vi "Step Response.vi"() -> ()   [LabVIEW 2020]
uses:
  <vilib>/addons/Control Design/_Model Construction/Data Typedefs.llb/CD Parametric Time Response Data.ctl
  <vilib>/addons/Control Design/_Model Construction/Model Creation.llb/Model Creation SubVI/cd_Create Transfer Function Model.vi
  <vilib>/addons/Control Design/_Dynamic Analysis/Dynamic Analysis.llb/Dynamic Analysis subVI/cd_Pole-Zero Map (Transfer Function).vi
  <vilib>/addons/Control Design/_Time Response Analysis/Time Response.llb/Time Response subVI/cd_Parametric Time Response (TF).vi
  <vilib>/addons/Control Design/_Time Response Analysis/Time Response.llb/Time Response subVI/cd_Step Response (Transfer Function).vi
  <vilib>/addons/Control Design/_Utility/Model Viewer.llb/Model Viewer SubVI/cd_Draw Transfer Function Equation (TF).vi
  <vilib>/addons/Control Design/_Model Construction/NI_LinSys_Model Creation.lvlib
  <vilib>/addons/Control Design/_Utility/NI_CD_Model Viewer.lvlib
  <vilib>/addons/Control Design/_Time Response Analysis/NI_CD_Time Response.lvlib
  <vilib>/addons/Control Design/_Dynamic Analysis/NI_CD_Dynamic Analysis.lvlib
  <vilib>/addons/Control Design/_Model Construction/NI_LinSys_Data Typedefs.lvlib
panel:
  out "Poles":cdb[](array[numeric])=[-3.2900000000000005-9.817122796420549i, -3.2900000000000005+9.817122796420549i] format="%.4f"
  out "Pole-Zero Map":cluster{dbl[], dbl[]}[](graph)=[{[-3.2900000000000005, -3.2900000000000005], [-9.817122796420549, 9.817122796420549]}, {[], []}]
  out "Time Response Parametric Data":T1={"Rise Time (s)"=[[0.12223540693995756]], "Peak Time (s)"=[[0.3259610851732202]], "Settling Time (s)"=[[1.3649620441628596]], "Overshoot (%)"=[[34.829275058539785]], "Steady-State Gain"=[[0.9999999999999999]], "Peak Value"=[[1.3482927505853977]]}
  out "Step Response Graph":cluster{"time":dbl[], dbl[]}[](graph)=[{"time"=[0.0, 0.020372567823326262, 0.040745135646652525, 0.06111770346997879, 0.08149027129330505, 0.10186283911663131, 0.12223540693995757, 0.14260797476328385, 0.1629805425866101, 0.18335311040993635, 0.20372567823326262, 0.2240982460565889, 0.24447081387991515, 0.2648433817032414, 0.2852159495265677, 0.30558851734989395, 0.3259610851732202, 0.34633365299654645, 0.3667062208198727, 0.387078788643199, 0.40745135646652525, 0.4278239242898515, 0.4481964921131778, 0.46856905993650405, 0.4889416277598303, 0.5093141955831566, 0.5296867634064828, 0.5500593312298091, 0.5704318990531354, 0.5908044668764616, 0.6111770346997879, 0.6315496025231141, 0.6519221703464404, 0.6722947381697667, 0.6926673059930929, 0.7130398738164192, 0.7334124416397454, 0.7537850094630717, 0.774157577286398, 0.7945301451097242, 0.8149027129330505, 0.8352752807563768, 0.855647848579703, 0.8760204164030293, 0.8963929842263556, 0.9167655520496818, 0.9371381198730081, 0.9575106876963343, 0.9778832555196606, 0.9982558233429869, 1.0186283911663132, 1.0390009589896394, 1.0593735268129656, 1.079746094636292, 1.1001186624596182, 1.1204912302829444, 1.1408637981062708, 1.161236365929597, 1.1816089337529232, 1.2019815015762494, 1.2223540693995758, 1.242726637222902, 1.2630992050462282, 1.2834717728695546, 1.3038443406928808, 1.324216908516207, 1.3445894763395334, 1.3649620441628596, 1.3853346119861858, 1.4057071798095122, 1.4260797476328384, 1.4464523154561646, 1.4668248832794908, 1.4871974511028172, 1.5075700189261434, 1.5279425867494696, 1.548315154572796, 1.5686877223961222, 1.5890602902194484, 1.6094328580427748, 1.629805425866101, 1.6501779936894272, 1.6705505615127536, 1.6909231293360798, 1.711295697159406, 1.7316682649827324, 1.7520408328060586, 1.7724134006293848, 1.7927859684527112, 1.8131585362760374, 1.8335311040993636, 1.8539036719226898, 1.8742762397460162, 1.8946488075693424, 1.9150213753926686, 1.935393943215995, 1.9557665110393212, 1.9761390788626474, 1.9965116466859738, 2.0168842145092998, 2.0372567823326264, 2.0576293501559526, 2.078001917979279, 2.098374485802605, 2.118747053625931, 2.1391196214492574, 2.159492189272584, 2.17986475709591, 2.2002373249192364, 2.2206098927425626, 2.240982460565889, 2.261355028389215, 2.2817275962125416, 2.302100164035868, 2.322472731859194, 2.34284529968252, 2.3632178675058464, 2.3835904353291726, 2.403963003152499, 2.4243355709758254, 2.4447081387991516], [0.0, 0.021206529908385886, 0.0803579450181118, 0.17023996814127196, 0.2832685265368125, 0.41185077065499803, 0.5487011653920958, 0.6871051771533931, 0.8211261920054864, 0.9457542028387028, 1.0569974026043463, 1.151920046588511, 1.228631753818595, 1.286234783637049, 1.324736746903471, 1.3449367094077282, 1.3482927505853977, 1.3367787984006523, 1.3127380249746132, 1.2787393163284961, 1.2374423849463327, 1.1914760366920671, 1.1433329919115829, 1.0952835472724662, 1.0493092964249129, 1.0070571426102635, 0.9698129652832004, 0.9384935674968039, 0.9136549447014484, 0.8955144843230233, 0.8839844274831129, 0.878713791806452, 0.8791359546581217, 0.8845192126858393, 0.8940178468071509, 0.9067215107945986, 0.9217011048811921, 0.9380496722865299, 0.9549172464662433, 0.9715389623548003, 0.9872561104693424, 1.0015301457960157, 1.0139499541562504, 1.024232920489682, 1.0322205323162654, 1.03786938635736, 1.0412385481036162, 1.0424742462602783, 1.041792871375323, 1.0394631967028252, 1.0357886564453616, 1.031090409365936, 1.0256917918487543, 1.0199046310619853, 1.0140177526633454, 1.008287884491235, 1.002933033014458, 0.9981282970993355, 0.9940039869869458, 0.9906458373148409, 0.9880970426377184, 0.9863618023617059, 0.9854100386668441, 0.9851829445370557, 0.9855990275958835, 0.98656033681754, 0.9879585908548885, 0.9896809660926718, 0.9916153469971529, 0.9936548884084502, 0.995701786828602, 0.9976702034884964, 0.999488324343489, 1.0010995798151614, 1.0024630790921285, 1.0035533395103557, 1.0043594106754505, 1.0048835055954362, 1.0051392574595954, 1.0051497213456588, 1.0049452357547293, 1.004561250273703, 1.0040362137343097, 1.0034096028891155, 1.0027201557565202, 1.002004357247872, 1.001295208250576, 1.0006212936709422, 1.0000061505931361, 0.9994679251151578, 0.9990192958820837, 0.9986676340302997, 0.9984153632484912, 0.9982604799125784, 0.9981971916346712, 0.9982166328801497, 0.9983076182968342, 0.9984573977731431, 0.9986523816846579, 0.9988788099821774, 0.9991233444094388, 0.9993735689260589, 0.9996183890917026, 0.9998483265188083, 1.000055709342634, 1.0002347638521012, 1.0003816158799894, 1.0004942132159464, 1.0005721821691043, 1.0006166324920656, 1.000629925237343, 1.0006154178270508, 1.0005771997703765, 1.0005198311658987, 1.0004480944876402, 1.000366768285526, 1.000280429439036, 1.0001932885854388, 1.0001090613879706, 1.0000308764881083, 0.9999612193583485]}]
  out "Equation":picture
  in  "Numerator":dbl[](array[numeric])=[107.2, 0.0, 0.0] format="%#.5g"
  in  "Denominator":dbl[](array[numeric])=[107.2, 6.58, 1.0, 0.0] format="%#.5g"
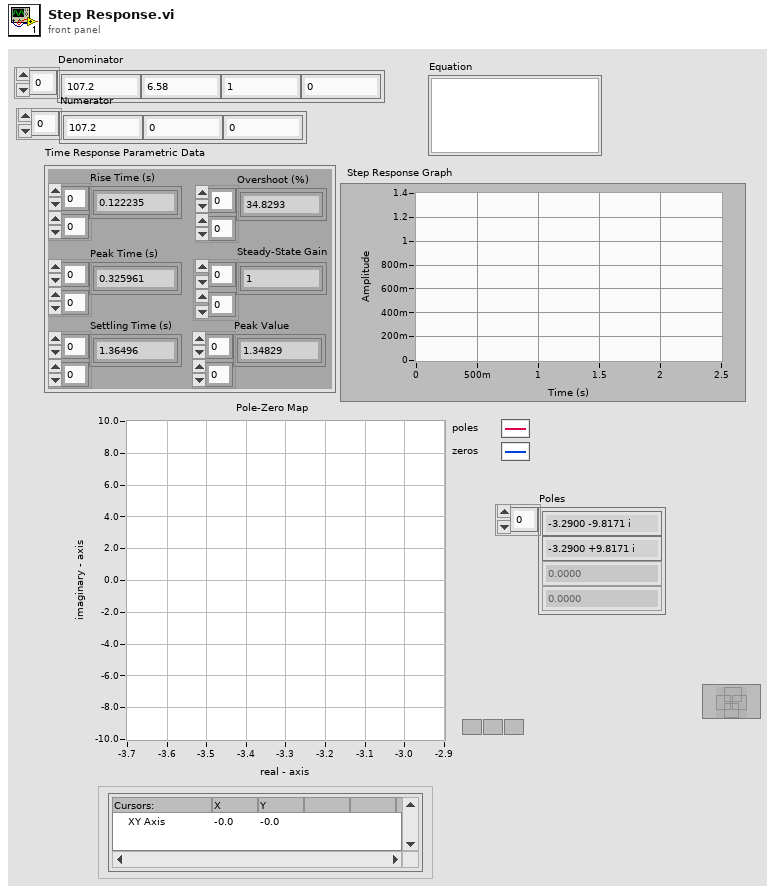
[diagram p1: front panel]
types:
  T1 = typedef "NI_LinSys_Data Typedefs.lvlib/CD Parametric Time Response Data.ctl" = cluster{"Rise Time (s)":dbl[][], "Peak Time (s)":dbl[][], "Settling Time (s)":dbl[][], "Overshoot (%)":dbl[][], "Steady-State Gain":dbl[][], "Peak Value":dbl[][]}
  T2 = typedef "NI_LinSys_Model Typedefs.lvlib/CD Transfer Function Model (MIMO).ctl" = cluster{"properties":T3, "transfer function(s)":T4[][]}
  T3 = typedef "NI_LinSys_Model Typedefs.lvlib/CD General Elements.ctl" = cluster{"Model name":string, "Input names":string[], "Output names":string[], "Input Delays":dbl[], "Output Delays":dbl[], "Sampling Time":dbl, "Notes":string}
  T4 = typedef "NI_LinSys_Model Typedefs.lvlib/CD Transfer Function Model (SISO).ctl" = cluster{"Numerator":dbl[], "Denominator":dbl[], "delay":dbl}
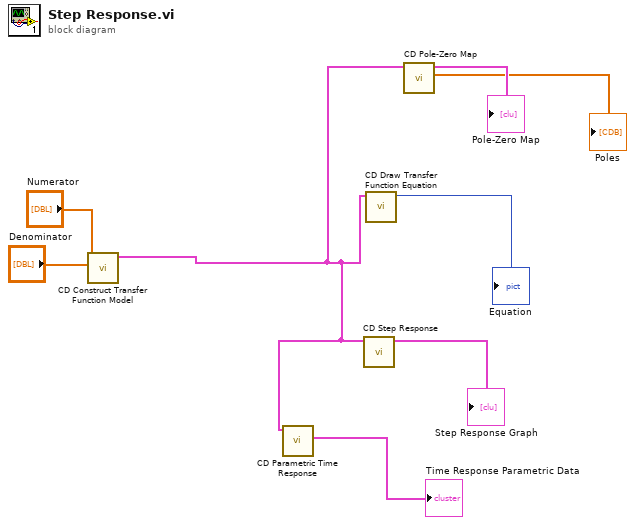
[diagram p0: block diagram]
diagram:
  n1 = call-poly <vilib>:"CD Construct Transfer Function Model.vi"("Denominator"="Denominator", "Numerator"="Numerator") -> ("Transfer Function Model"=w3:T2)  [unwired: 8 in, 1 out]
  n2 = call-poly <vilib>:"CD Parametric Time Response.vi"("Transfer Function Model"=w3) -> ("Time Response Parametric Data"=→"Time Response Parametric Data":T1)  [unwired: 7 in, 3 out]
  n3 = call-poly <vilib>:"CD Step Response.vi"("Transfer Function Model"=w3) -> ("Step Response Graph"=→"Step Response Graph":cluster{"time":dbl[], dbl[]}[])  [unwired: 8 in, 2 out]
  n4 = call-poly <vilib>:"CD Draw Transfer Function Equation.vi"("Transfer Function Model"=w3) -> ("Equation"=→"Equation":picture)  [unwired: 8 in, 2 out]
  n5 = call-poly <vilib>:"CD Pole-Zero Map.vi"("Transfer Function Model"=w3) -> ("Poles"=→"Poles":cdb[], "Pole-Zero Map"=→"Pole-Zero Map":cluster{dbl[], dbl[]}[])  [unwired: 7 in, 2 out]
